vi "DriverStation Get Remaining Match Time.vi"(8 "error in (no error)":errorcluster) -> (0 "error out":errorcluster, 2 "OutputsEnabled?":bool, 3 "Match Time(s)":sgl)   [LabVIEW 2023, in "MrcLib.lvlib"]
doc: "Returns the time remaining in the current portion of the robot match. It returns -1 if the robot is disabled or in an untimed mode."
uses:
  <vilib>/MRC/MrcLib.lvlib
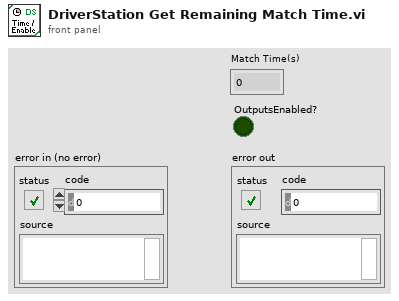
[diagram p1: front panel]
types:
  T1 = typedef "MrcLib.lvlib/MRC_ControlData.ctl" = cluster{"controlFlags":u32, "matchTime":u16, "currentOpMode":u64, "gameDataLength":u8, "game data":T2}
  T2 = typedef "MRC Str64.ctl" = cluster{"[0]":u8, "[1]":u8, "[2]":u8, "[3]":u8, "[4]":u8, "[5]":u8, "[6]":u8, "[7]":u8, "[8]":u8, "[9]":u8, "[10]":u8, "[11]":u8, "[12]":u8, "[13]":u8, "[14]":u8, "[15]":u8, "[16]":u8, "[17]":u8, "[18]":u8, "[19]":u8, "[20]":u8, "[21]":u8, "[22]":u8, "[23]":u8, "[24]":u8, "[25]":u8, "[26]":u8, "[27]":u8, "[28]":u8, "[29]":u8, "[30]":u8, "[31]":u8, "[32]":u8, "[33]":u8, "[34]":u8, "[35]":u8, "[36]":u8, "[37]":u8, "[38]":u8, "[39]":u8, "[40]":u8, "[41]":u8, "[42]":u8, "[43]":u8, "[44]":u8, "[45]":u8, "[46]":u8, "[47]":u8, "[48]":u8, "[49]":u8, "[50]":u8, "[51]":u8, "[52]":u8, "[53]":u8, "[54]":u8, "[55]":u8, "[56]":u8, "[57]":u8, "[58]":u8, "[59]":u8, "[60]":u8, "[61]":u8, "[62]":u8, "[63]":u8}
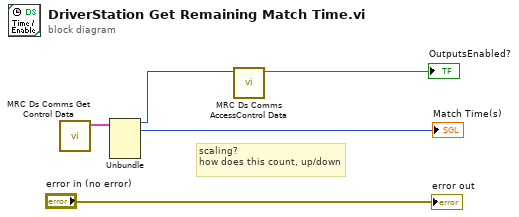
[diagram p0: block diagram]
diagram:
  # "scaling?\nhow does this count, up/down"
  n1 = call <vilib>:"MRC Ds Comms Get Control Data.vi"() -> ("data out"=w4:T1)  [unwired: 10 in, 1 out]
  n2 = Unbundle(w4) -> ("controlFlags"=w1:u32, "matchTime"=→"Match Time(s)":u16)  [unwired: 3 out]
  n3 = call <vilib>:"MRC Ds Comms AccessControl Data.vi"("controlFlag"=w1) -> ("Enabled"=→"OutputsEnabled?":bool)  [unwired: 7 in, 3 out]
  "error out" <- "error in (no error)"
